vi "Test Server Reopen Same Port.vi"(8 "error in (no error)":errorcluster) -> (0 "error out":errorcluster)   [LabVIEW 2019, in "RemoteControl.ZMQ.Tests.lvclass"]
uses:
  RemoteControl.ZMQ.Tests.lvclass
  <vilib>/addons/_JKI Toolkits/Caraya/classes/Assert/Assert Not Error.vi
  <vilib>/addons/_JKI Toolkits/Caraya/classes/Assert/Assert.lvclass
  <vilib>/addons/_JKI Toolkits/Caraya/classes/Test/Test.lvclass
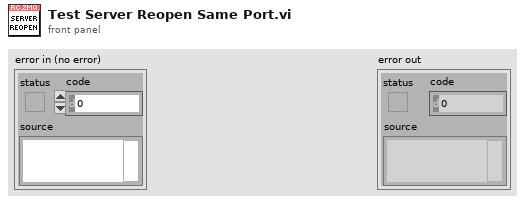
[diagram p1: front panel]
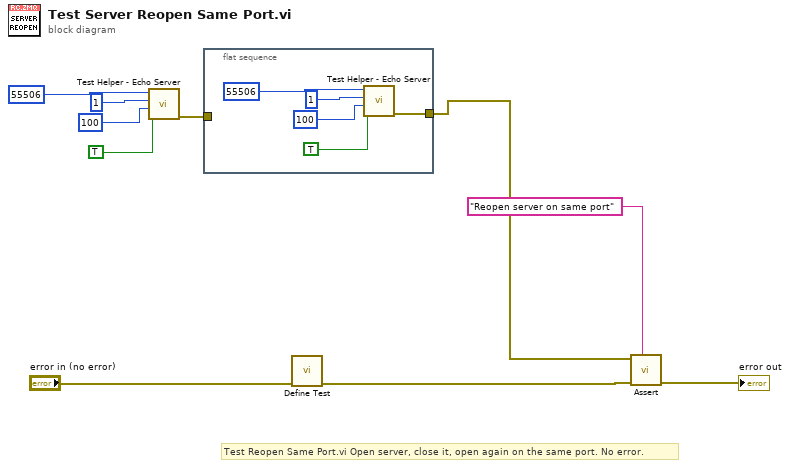
[diagram p0: block diagram]
diagram:
  # "Test Reopen Same Port.vi\tOpen server, close it, open again on the same port.\tNo error."
  n1 = call "Test Helper - Echo Server.vi"("Answer?"=TRUE, "reply delay (ms)"=u32 100, "number of messages"=1, "port"=u16 55506 ("Port")) -> ("error out"=w2:errorcluster)  [unwired: 6 in, 1 out]
  n2 = flat-sequence {
    tunnel: w2 -> [_]
    tunnel: [w11] -> w4
    frame #0 {
      n3 = call "Test Helper - Echo Server.vi"("Answer?"=TRUE, "reply delay (ms)"=u32 100, "number of messages"=1, "port"=u16 55506 ("Port")) -> ("error out"=w11:errorcluster)  [unwired: 6 in, 1 out]
    }
  }
  n4 = call <vilib>:"Define Test.vi"("error in (no error)"="error in (no error)") -> ("error out"=w1:errorcluster)  [unwired: 9 in, 1 out]
  n5 = call-poly <vilib>:"Assert.vi"("Label"="Reopen server on same port", "error in (no error)"=w1, "Not Error?"=w4) -> ("error out"=→"error out":errorcluster)  [unwired: 7 in, 1 out]
